vi "device class selection.vi"(3 "detect all (F)":bool, 7 "device classes":T2) -> (1 "device class":T1[](array[typedef]))   [LabVIEW 2014, in "SMI.lvlib" / "Device.lvclass"]
uses:
  Device.lvclass
  device class selection.ctl
  device class.ctl
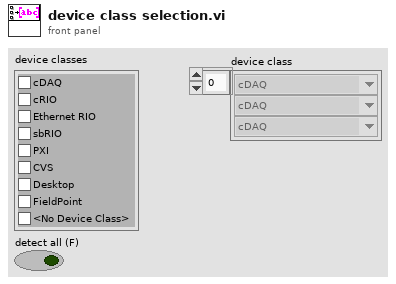
[diagram p1: front panel]
types:
  T1 = typedef "SMI.lvlib/Device.lvclass/device class.ctl" = enum16{"cDAQ", "cRIO", "Ethernet RIO", "sbRIO", "PXI", "CVS", "Desktop", "FieldPoint", "<No Device Class>", "<Detect All>"}
  T2 = typedef "SMI.lvlib/Device.lvclass/device class selection.ctl" = cluster{"cDAQ":bool, "cRIO":bool, "Ethernet RIO":bool, "sbRIO":bool, "PXI":bool, "CVS":bool, "Desktop":bool, "FieldPoint":bool, "<No Device Class>":bool}
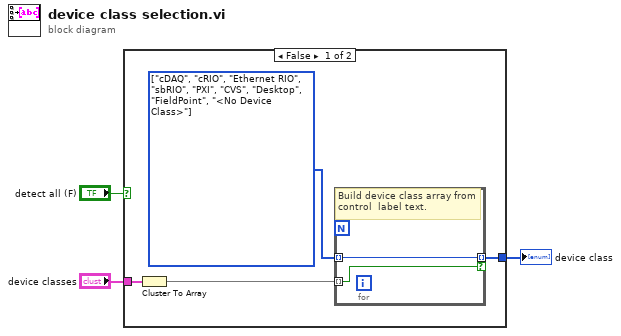
[diagram p0: block diagram]
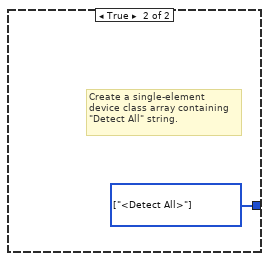
[diagram p2: hidden frame]
diagram:
  n1 = case shown="False" "detect all (F)" {
    tunnel: "device classes" -> [w7 _]
    tunnel: [w4 w10] -> w2
    frame False {
      w5 = T1[] [enum."cDAQ", enum."cRIO", enum."Ethernet RIO", enum."sbRIO", enum."PXI", enum."CVS", enum."Desktop", enum."FieldPoint", enum."<No Device Class>"] items=["cDAQ", "cRIO", "Ethernet RIO", "sbRIO", "PXI", "CVS", "Desktop", "FieldPoint", "<No Device Class>", "<Detect All>"]
      n2 = Cluster To Array(cluster=w7) -> (array=w6:bool[])
      n3 = for {
        tunnel: w6 -> [w9] mode=indexing
        tunnel: [w8] -> w4 mode=indexing if=w9
        tunnel: w5 -> [w8] mode=indexing
        # "Build device class array from control  label text."
      }
    }
    frame True {
      w10 = T1[] [enum."<Detect All>"] items=["cDAQ", "cRIO", "Ethernet RIO", "sbRIO", "PXI", "CVS", "Desktop", "FieldPoint", "<No Device Class>", "<Detect All>"]
      # "Create a single-element\ndevice class array containing\n\"Detect All\" string."
    }
  }
  "device class" <- w2
